vi "Init.vi"(8 "error in (no error)":errorcluster, 11 "WEG_SCA06_Modbus in":refnum<class "WEG_SCA06_Modbus.lvclass">) -> (0 "error out":errorcluster, 3 "WEG_SCA06_Modbus out":refnum<class "WEG_SCA06_Modbus.lvclass">)   [LabVIEW 2021, in "WEG_SCA06_Modbus.lvclass"]
uses:
  WEG_SCA06_Modbus.lvclass
  C:/Users/lincoln.lucio/Documents/Lincoln/Documentos Pessoais/meus docs/Projetos pessoais/Projeto Sciranda/projeto_versioned/sciranda/ServoDrive/ServoDrive.lvclass
  WEG_SCA06_Modbus.lvclass/WEG_SCA06_Modbus.ctl
  ServoDrive/ServoDrive.lvclass/ServoDrive.ctl
  ServoDrive/Accessor VIs/Read Accel_ms_krpm.vi
  ServoDrive/Accessor VIs/Read Decel_ms_krpm.vi
  Modbus_Master/Modbus_Master.lvclass
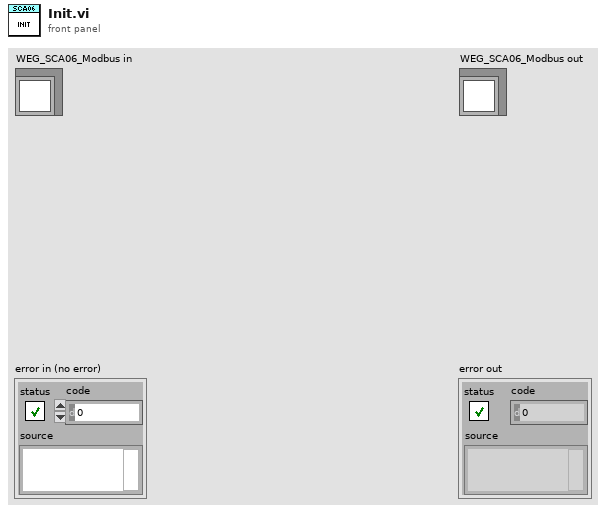
[diagram p1: front panel]
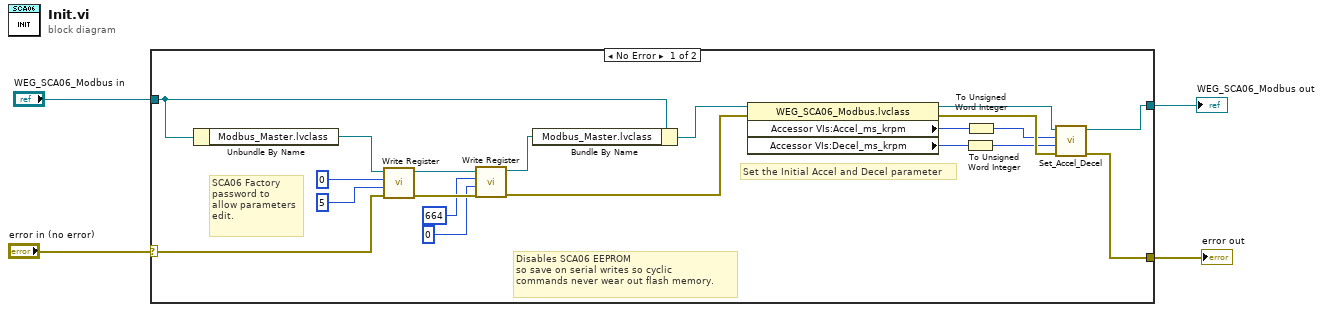
[diagram p0: block diagram]
diagram:
  n1 = case shown="No Error" "error in (no error)" {
    selector: "error in (no error)" -> [w23 w26]
    tunnel: "WEG_SCA06_Modbus in" -> [w15 w25]
    tunnel: [w8 w25] -> w2
    tunnel: [w7 w26] -> w1
    frame No Error {
      # "Set the Initial Accel and Decel parameter"
      # "SCA06 Factory\npassword to \nallow parameters\nedit."
      # "Disables SCA06 EEPROM\nso save on serial writes so cyclic\ncommands never wear out flash memory."
      n2 = Unbundle By Name(w15) -> ("Modbus_Master.lvclass"=w24:refnum<class "Modbus_Master.lvclass">)
      n3 = call "Write Register.vi"("error in (no error)"=w23, "Value"=u16 5, "Register Address"=u16 0, "Modbus_Master in"=w24) -> ("error out"=w19:errorcluster, "Modbus_Master out"=w20:refnum<class "Modbus_Master.lvclass">)  [unwired: 6 in]
      n4 = call "Write Register.vi"("error in (no error)"=w19, "Value"=u16 0, "Register Address"=u16 664, "Modbus_Master in"=w20) -> ("error out"=w13:errorcluster, "Modbus_Master out"=w16:refnum<class "Modbus_Master.lvclass">)  [unwired: 6 in]
      n5 = Bundle By Name(cluster=w15, "Modbus_Master.lvclass"=w16) -> (w14:refnum<class "WEG_SCA06_Modbus.lvclass">)
      n6 = property class="WEG_SCA06_Modbus.lvclass"(reference=w14, error in=w13) -> (reference out=w12:refnum<class "WEG_SCA06_Modbus.lvclass">, error out=w9:errorcluster, "Accessor VIs:Accel_ms_krpm"=w11:i32, "Accessor VIs:Decel_ms_krpm"=w10:i32)
      n7 = To Unsigned Word Integer(number=w10) -> (unsigned 16bit integer=w5:u16)
      n8 = To Unsigned Word Integer(number=w11) -> (unsigned 16bit integer=w6:u16)
      n9 = call-dynamic "Set_Accel_Decel.vi"("error in (no error)"=w9, "Decel (ms/krpm)"=w5, "Accel (ms/krpm)"=w6, "WEG_SCA06_Modbus in"=w12) -> ("error out"=w7:errorcluster, "WEG_SCA06_Modbus out"=w8:refnum<class "WEG_SCA06_Modbus.lvclass">)  [unwired: 6 in]
    }
    frame Error {
    }
  }
  "error out" <- w1
  "WEG_SCA06_Modbus out" <- w2
